vi "test batch.vi"(8 "error in (no error)":errorcluster) -> (0 "error out":errorcluster, 3 "body":string)   [LabVIEW 2020, in "MCP Server tests.lvlib"]
doc: "A JSON array of messages is answered with a JSON array of the answers, without entries for notifications. A batch of notifications only is answered with 202 and no body. An empty batch is an invalid request."
uses:
  MCP Server tests.lvlib
  <vilib>/JDP Science/JSONtext/Next JSON Value.vi
  <vilib>/JDP Science/JSONtext/String Subset.vi
  <vilib>/JDP Science/JSONtext/Parsing/Advance past next JSON Value (inlined COPY).vi
  <vilib>/JDP Science/JSONtext/Parsing/Advance past whitespace.vi
  <vilib>/JDP Science/JSONtext/Parsing/Advance past String.vi
  <vilib>/JDP Science/JSONtext/Parsing/Advance past Number.vi
  <vilib>/JDP Science/JSONtext/Parsing/Advance past Line Ending.vi
  <vilib>/JDP Science/JSONtext/Parsing/Parse Full Path or Item Name.vi
  <vilib>/JDP Science/JSONtext/Parsing/Advance past Array.vi
  <vilib>/JDP Science/JSONtext/Parsing/Advance past Object.vi
  <vilib>/JDP Science/JSONtext/support/Error Cluster From Code.vi
  <vilib>/JDP Science/JSONtext/Offset/Find Item Locations by Path.vi
  <vilib>/addons/_JKI Toolkits/Caraya/classes/Test/Test.lvclass
  <vilib>/JDP Science/JSONtext/JSONtext.lvlib
  <vilib>/addons/_JKI Toolkits/Caraya/classes/Assert/Assert.lvclass
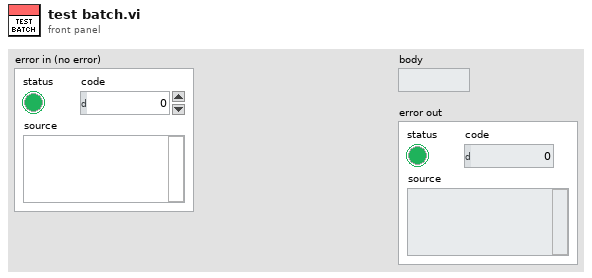
[diagram p1: front panel]
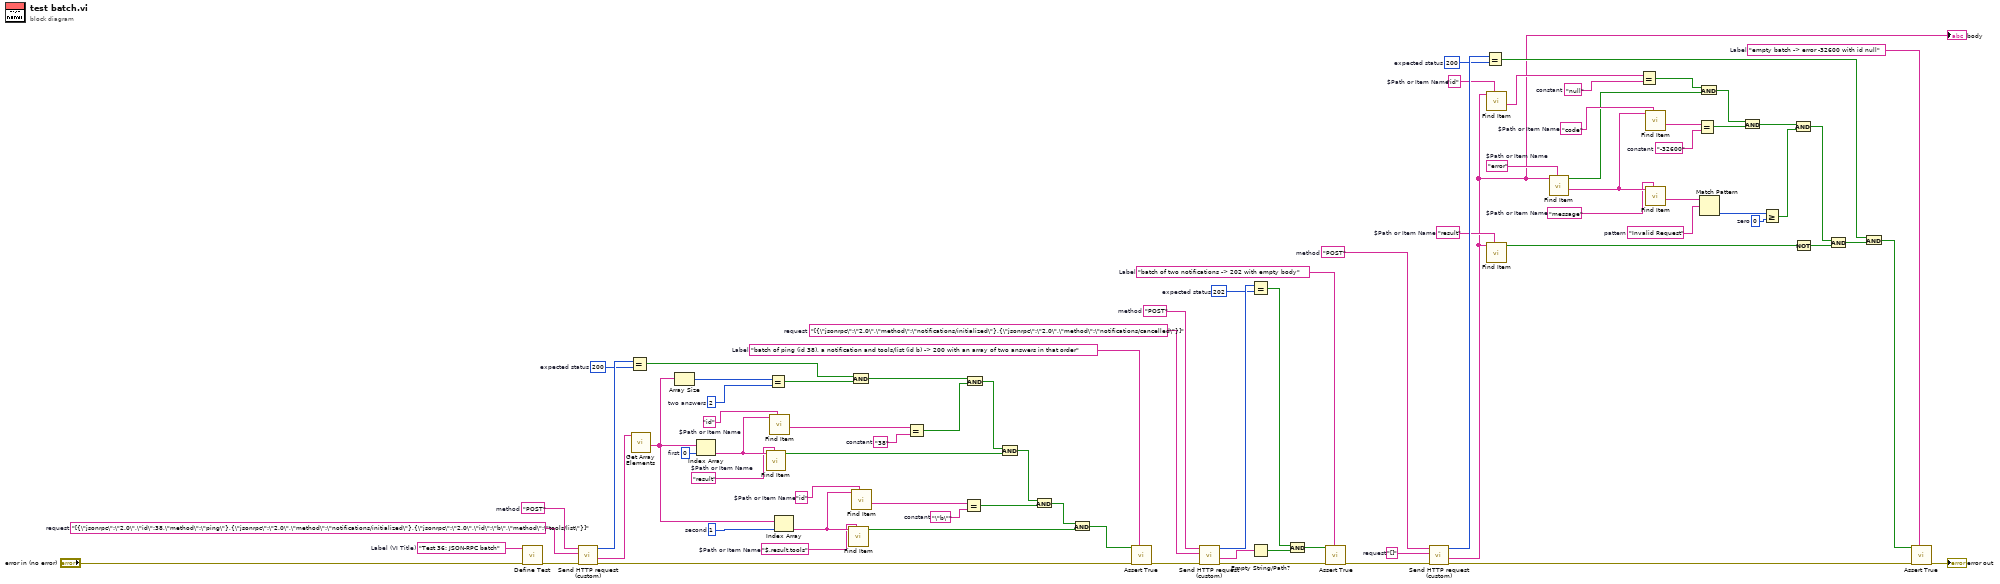
[diagram p0: block diagram]
diagram:
  w3 = "empty batch -> error -32600 with id null"  # Label
  w17 = 0  # zero
  w19 = "Invalid Request"  # pattern
  w21 = "-32600"  # constant
  w23 = "null"  # constant
  w25 = "result"  # $Path or Item Name
  w26 = "message"  # $Path or Item Name
  w28 = "code"  # $Path or Item Name
  w29 = "error"  # $Path or Item Name
  w30 = "id"  # $Path or Item Name
  w31 = 200  # expected status
  w34 = "[]"  # request
  w35 = "POST"  # method
  w36 = "batch of two notifications -> 202 with empty body"  # Label
  w42 = 202  # expected status
  w45 = "[{\"jsonrpc\":\"2.0\",\"method\":\"notifications/initialized\"},{\"jsonrpc\":\"2.0\",\"method\":\"notifications/cancelled\"}]"  # request
  w46 = "POST"  # method
  w47 = "batch of ping (id 38), a notification and tools/list (id b) -> 200 with an array of two answers in that order"  # Label
  w60 = "\"b\""  # constant
  w62 = "38"  # constant
  w64 = 2  # two answers
  w66 = "$.result.tools"  # $Path or Item Name
  w68 = "id"  # $Path or Item Name
  w69 = "result"  # $Path or Item Name
  w71 = "id"  # $Path or Item Name
  w72 = 1  # second
  w74 = 0  # first
  w76 = 200  # expected status
  w79 = "[{\"jsonrpc\":\"2.0\",\"id\":38,\"method\":\"ping\"},{\"jsonrpc\":\"2.0\",\"method\":\"notifications/initialized\"},{\"jsonrpc\":\"2.0\",\"id\":\"b\",\"method\":\"tools/list\"}]"  # request
  w80 = "POST"  # method
  w82 = "Test 36: JSON-RPC batch"  # Label (VI Title)
  n1 = call <vilib>:"Define Test.vi"("error in (no error)"="error in (no error)", "Label (VI Title)"=w82) -> ("error out"=w78:errorcluster)  [unwired: 8 in, 1 out]
  n2 = call "Send HTTP request (custom).vi"("error in (no error)"=w78, "request"=w79, "method"=w80) -> ("error out"=w48:errorcluster, "response"=w75:string, "status code"=w77:i32)  [unwired: 5 in, 1 out]
  n3 = Equal?(x=w77, y=w76) -> (x = y?=w59:bool)
  n4 = call <vilib>:"Get Array Elements.vi"("JSON"=w75) -> ("<JSON>"=w73:string[])  [unwired: 8 in, 2 out]
  n5 = Array Size(array=w73) -> (size(s)=w65:i32)
  n6 = Index Array(array=w73, index=w74) -> (element=w70:string)
  n7 = call <vilib>:"Find Item.vi"("$Path or Item Name"=w69, "JSON"=w70) -> ("Found"=w54:bool)  [unwired: 6 in, 3 out]
  n8 = Equal?(x=w65, y=w64) -> (x = y?=w58:bool)
  n9 = call <vilib>:"Find Item.vi"("$Path or Item Name"=w71, "JSON"=w70) -> ("<JSON>"=w63:string)  [unwired: 6 in, 3 out]
  n10 = Index Array(array=w73, index=w72) -> (element=w67:string)
  n11 = call <vilib>:"Find Item.vi"("$Path or Item Name"=w66, "JSON"=w67) -> ("Found"=w50:bool)  [unwired: 6 in, 3 out]
  n12 = And(x=w59, y=w58) -> (x .and. y?=w57:bool)
  n13 = call <vilib>:"Find Item.vi"("$Path or Item Name"=w68, "JSON"=w67) -> ("<JSON>"=w61:string)  [unwired: 6 in, 3 out]
  n14 = Equal?(x=w63, y=w62) -> (x = y?=w56:bool)
  n15 = Equal?(x=w61, y=w60) -> (x = y?=w52:bool)
  n16 = And(x=w57, y=w56) -> (x .and. y?=w55:bool)
  n17 = And(x=w55, y=w54) -> (x .and. y?=w53:bool)
  n18 = And(x=w53, y=w52) -> (x .and. y?=w51:bool)
  n19 = And(x=w51, y=w50) -> (x .and. y?=w49:bool)
  n20 = call <vilib>:"Assert True.vi"("Label"=w47, "error in (no error)"=w48, "True?"=w49) -> ("error out"=w44:errorcluster)  [unwired: 7 in, 1 out]
  n21 = call "Send HTTP request (custom).vi"("error in (no error)"=w44, "request"=w45, "method"=w46) -> ("error out"=w37:errorcluster, "response"=w41:string, "status code"=w43:i32)  [unwired: 5 in, 1 out]
  n22 = Equal?(x=w43, y=w42) -> (x = y?=w40:bool)
  n23 = Empty String/Path?(string/path=w41) -> (empty?=w39:bool)
  n24 = And(x=w40, y=w39) -> (x .and. y?=w38:bool)
  n25 = call <vilib>:"Assert True.vi"("Label"=w36, "error in (no error)"=w37, "True?"=w38) -> ("error out"=w33:errorcluster)  [unwired: 7 in, 1 out]
  n26 = call "Send HTTP request (custom).vi"("error in (no error)"=w33, "request"=w34, "method"=w35) -> ("error out"=w4:errorcluster, "response"=w2:string, "status code"=w32:i32)  [unwired: 5 in, 1 out]
  "body" <- w2
  n27 = Equal?(x=w32, y=w31) -> (x = y?=w7:bool)
  n28 = call <vilib>:"Find Item.vi"("$Path or Item Name"=w30, "JSON"=w2) -> ("<JSON>"=w24:string)  [unwired: 6 in, 3 out]
  n29 = call <vilib>:"Find Item.vi"("$Path or Item Name"=w25, "JSON"=w2) -> ("Found"=w16:bool)  [unwired: 6 in, 3 out]
  n30 = call <vilib>:"Find Item.vi"("$Path or Item Name"=w29, "JSON"=w2) -> ("<JSON>"=w27:string, "Found"=w14:bool)  [unwired: 6 in, 2 out]
  n31 = Equal?(x=w24, y=w23) -> (x = y?=w15:bool)
  n32 = call <vilib>:"Find Item.vi"("$Path or Item Name"=w28, "JSON"=w27) -> ("<JSON>"=w22:string)  [unwired: 6 in, 3 out]
  n33 = call <vilib>:"Find Item.vi"("$Path or Item Name"=w26, "JSON"=w27) -> ("<JSON>"=w20:string)  [unwired: 6 in, 3 out]
  n34 = Equal?(x=w22, y=w21) -> (x = y?=w12:bool)
  n35 = And(x=w15, y=w14) -> (x .and. y?=w13:bool)
  n36 = Match Pattern(string=w20, regular expression=w19) -> (offset past match=w18:i32)  [unwired: 1 in, 3 out]
  n37 = And(x=w13, y=w12) -> (x .and. y?=w11:bool)
  n38 = Greater Or Equal?(x=w18, y=w17) -> (x >= y?=w10:bool)
  n39 = And(x=w11, y=w10) -> (x .and. y?=w9:bool)
  n40 = Not(x=w16) -> (.not. x?=w8:bool)
  n41 = And(x=w9, y=w8) -> (x .and. y?=w6:bool)
  n42 = And(x=w7, y=w6) -> (x .and. y?=w5:bool)
  n43 = call <vilib>:"Assert True.vi"("Label"=w3, "error in (no error)"=w4, "True?"=w5) -> ("error out"=→"error out":errorcluster)  [unwired: 7 in, 1 out]
